vi "Ref to Error.vi"(11 "references":T1) -> (3 "error out":errorcluster)   [LabVIEW 2011]
doc: "Merge all errors from Measurement References cluster."
uses:
  Measurement References.ctl
  <vilib>/Utility/NIReport.llb/NI_report.lvclass
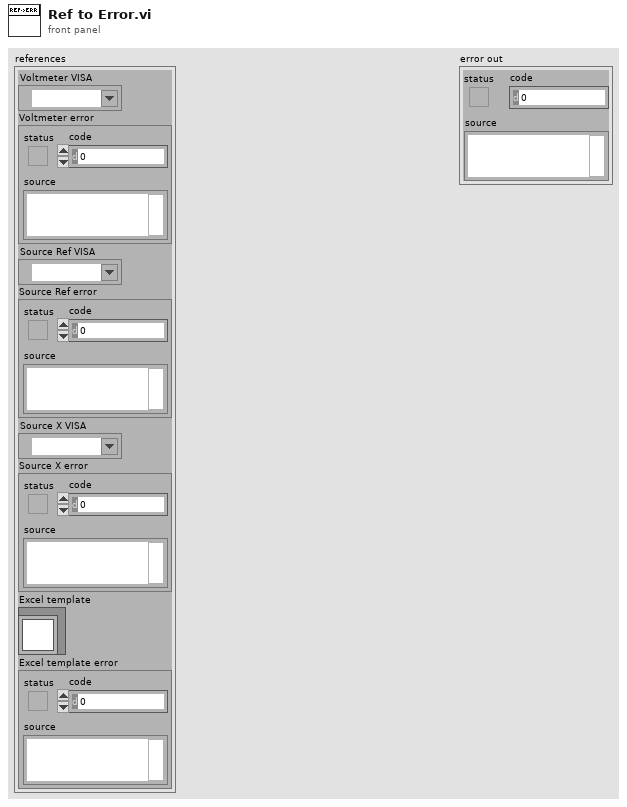
[diagram p1: front panel]
types:
  T1 = typedef "Measurement References.ctl" = cluster{"Voltmeter VISA":refnum<visa-resource-name>, "Voltmeter error":errorcluster, "Source Ref VISA":refnum<visa-resource-name>, "Source Ref error":errorcluster, "Source X VISA":refnum<visa-resource-name>, "Source X error":errorcluster, "Excel template":refnum<class "NI_report.lvclass">, "Excel template error":errorcluster}
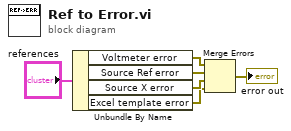
[diagram p0: block diagram]
diagram:
  n1 = Unbundle By Name("references") -> ("Voltmeter error"=w5:errorcluster, "Source Ref error"=w4:errorcluster, "Source X error"=w3:errorcluster, "Excel template error"=w2:errorcluster)
  n2 = Merge Errors(w5, w4, w3, w2) -> (→"error out":errorcluster)
